vi "Exp - Get Operand Value.vi"(4 "ena complex? (F)":bool, 5 "ena string? (F)":bool, 6 "error in":bool, 8 "op info":T2, 9 "InstanceRef":T1) -> (0 "error out":bool, 1 "type":u32=1, 2 "str":string, 3 "num":dbl=nan)   [LabVIEW 2021]
doc: "::: CalcExpress Toolkit :::\nCopyright (c) 2000-2026 Konstantin Shifershteyn. All rights reserved."
uses:
  cetypes.llb/CalcExpress Function Argument Info.ctl
  cetypes.llb/CalcExpress Instance RefNum.ctl
  cersrc/celveng32.dll
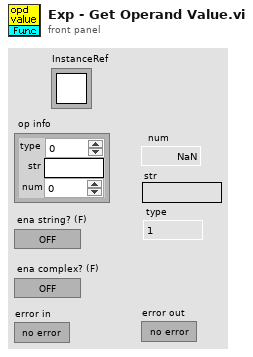
[diagram p1: front panel]
types:
  T1 = typedef "CalcExpress Instance RefNum.ctl" = refnum<k1>
  T2 = typedef "CalcExpress Function Argument Info.ctl" = cluster{"type":u32, "str":string, "num":dbl}
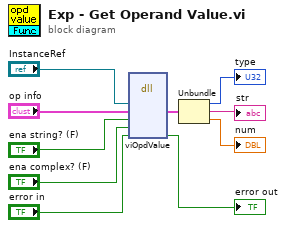
[diagram p0: block diagram]
diagram:
  n1 = dll-call lib="C:/LV Projects/CalcExpress 40 LV2021/vi.lib/addons/CalcExpress/cersrc/celveng*.dll" fn="viOpdValue"("iRef"="InstanceRef", "opd"="op info", "enStr"="ena string? (F)", "enNonDbl"="ena complex? (F)", "erf"="error in") -> ("opd"=w1:T2, "erf"=→"error out":bool)  [unwired: 7 in, 2 out]
  n2 = Unbundle(w1) -> ("type"=→"type":u32, "str"=→"str":string, "num"=→"num":dbl)
